vi "process.vi"(8 "error in":errorcluster, 9 "result allocation":T1, 10 "parameters":T1, 11 "module in":refnum<class "alarms module runtime.lvclass">) -> (0 "error out":errorcluster, 1 "results":T1, 2 "parameter allocation":T1, 3 "module out":refnum<class "alarms module runtime.lvclass">)   [LabVIEW 2013, in "alarms module runtime.lvclass"]
doc: "Provides an interface for information processing by a module at runtime. While this interface performs no operations, a child should provide an override which may process data in any manner necessary."
uses:
  alarms module runtime.lvclass
  <vilib>/NI/Tag Bus/table/data table.lvlib
  <vilib>/NI/Tag Bus/table/data polymorphs/read one/read Boolean.vi
  <vilib>/NI/Tag Bus/table/data polymorphs/write one/write Boolean.vi
  <vilib>/NI/Tag Bus/table/data polymorphs/read one/read Single.vi
  <vilib>/NI/Tag Bus/table/data polymorphs/read one/read Double.vi
  <vilib>/NI/Tag Bus/table/data polymorphs/read one/read I64.vi
  <vilib>/NI/Tag Bus/table/data polymorphs/read one/read I32.vi
  <vilib>/NI/Tag Bus/table/data polymorphs/read one/read I16.vi
  <vilib>/NI/Tag Bus/table/data polymorphs/read one/read I8.vi
  <vilib>/NI/Tag Bus/table/data polymorphs/read one/read U64.vi
  <vilib>/NI/Tag Bus/table/data polymorphs/read one/read U32.vi
  <vilib>/NI/Tag Bus/table/data polymorphs/read one/read U16.vi
  <vilib>/NI/Tag Bus/table/data polymorphs/read one/read U8.vi
  <vilib>/NI/Tag Bus/table/data table.ctl
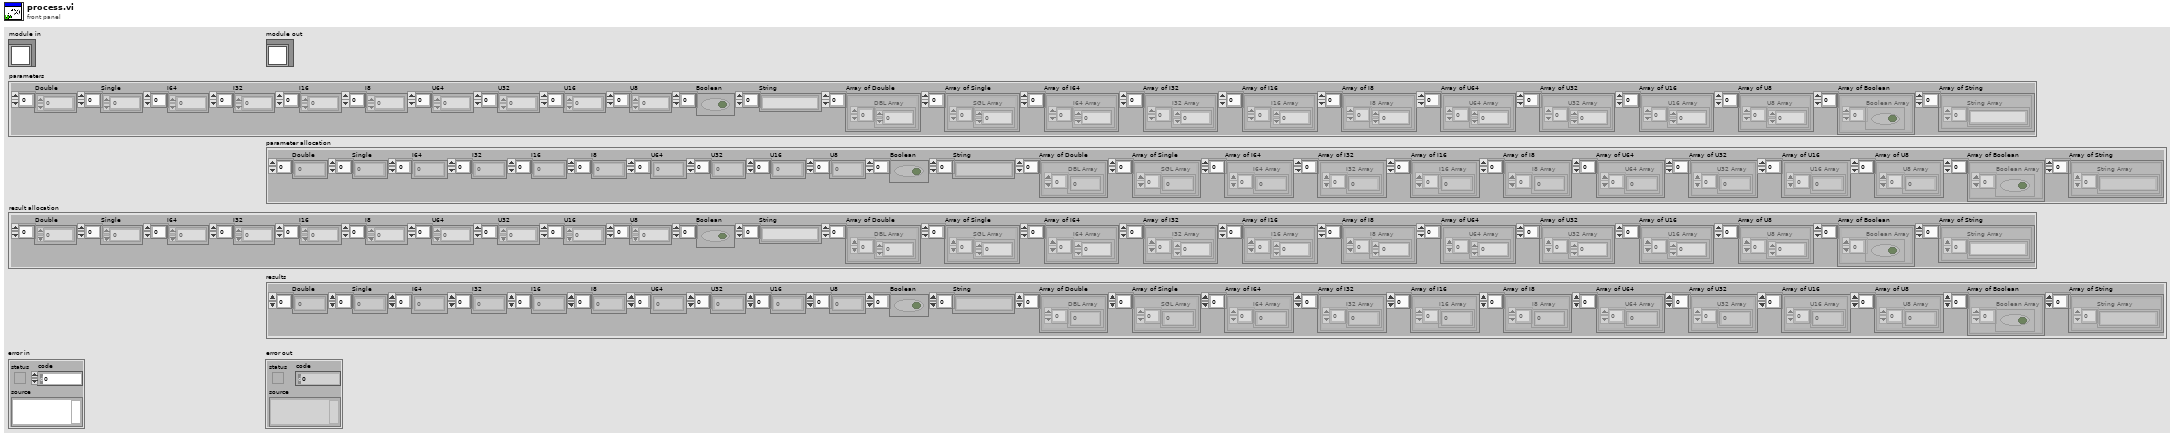
[diagram p1: front panel]
types:
  T1 = typedef "tag bus.lvlib/data table.lvlib/data table.ctl" = cluster{"Double":dbl[], "Single":sgl[], "I64":i64[], "I32":i32[], "I16":i16[], "I8":i8[], "U64":u64[], "U32":u32[], "U16":u16[], "U8":u8[], "Boolean":bool[], "String":string[], "Array of Double":cluster{"DBL Array":dbl[]}[], "Array of Single":cluster{"SGL Array":sgl[]}[], "Array of I64":cluster{"I64 Array":i64[]}[], "Array of I32":cluster{"I32 Array":i32[]}[], "Array of I16":cluster{"I16 Array":i16[]}[], "Array of I8":cluster{"I8 Array":i8[]}[], "Array of U64":cluster{"U64 Array":u64[]}[], "Array of U32":cluster{"U32 Array":u32[]}[], "Array of U16":cluster{"U16 Array":u16[]}[], "Array of U8":cluster{"U8 Array":u8[]}[], "Array of Boolean":cluster{"Boolean Array":bool[]}[], "Array of String":cluster{"String Array":string[]}[]}
  T2 = typedef "alarms module runtime.lvclass/runtime alarm configuration.ctl" = cluster{"comparisons":T3[], "boolean op":T6, "unlatch index (bool)":i32, "output index (bool)":i32, "state":bool}
  T3 = typedef "alarms module runtime.lvclass/runtime alarm comparison.ctl" = cluster{"data type":T4, "index":i32, "limit":dbl, "comparison":T5}
  T4 = typedef "tag bus.lvlib/tag descriptor.lvclass/Data Type.ctl" = enum16{"Double", "Single", "I64", "I32", "I16", "I8", "U64", "U32", "U16", "U8", "Boolean", "String", "Array of Double", "Array of Single", "Array of I64", "Array of I32", "Array of I16", "Array of I8", "Array of U64", "Array of U32", "Array of U16", "Array of U8", "Array of Boolean", "Array of String"}
  T5 = typedef "alarms module configuration.lvclass/compare type.ctl" = enum16{">", "<", ">=", "<=", "="}
  T6 = typedef "alarms module configuration.lvclass/boolean operation.ctl" = enum16{"AND", "OR"}
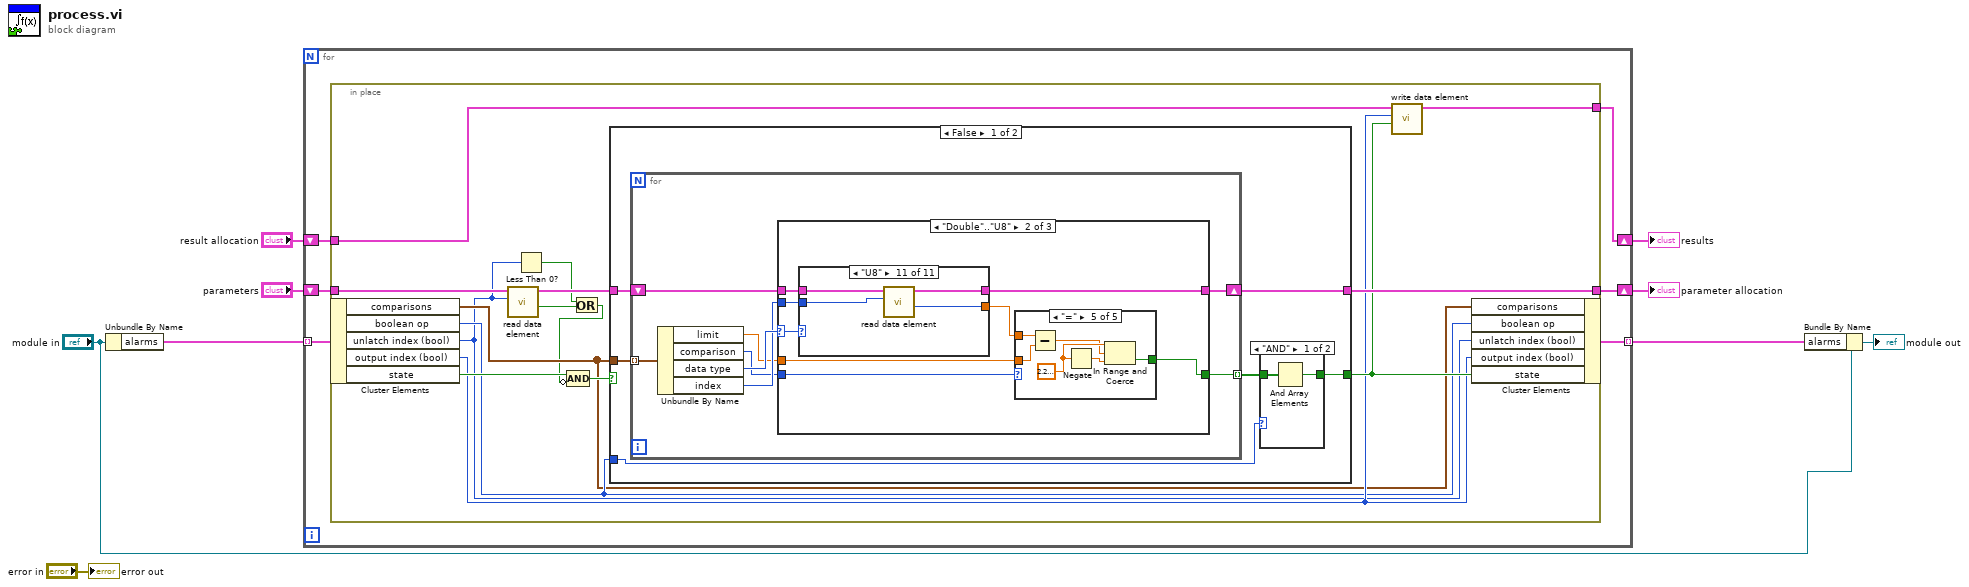
[diagram p0: block diagram]
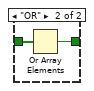
[diagram p2: hidden frame]
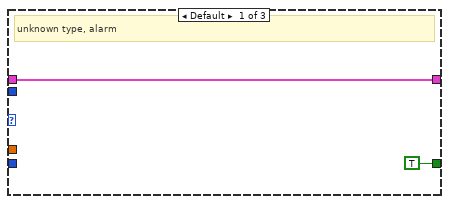
[diagram p3: hidden frame]
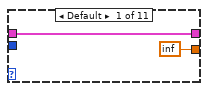
[diagram p4: hidden frame]
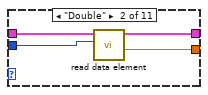
[diagram p5: hidden frame]
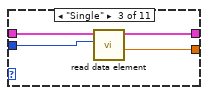
[diagram p6: hidden frame]
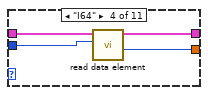
[diagram p7: hidden frame]
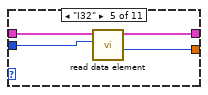
[diagram p8: hidden frame]
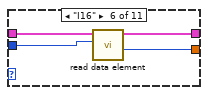
[diagram p9: hidden frame]
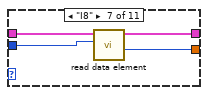
[diagram p10: hidden frame]
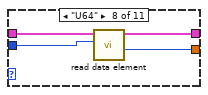
[diagram p11: hidden frame]
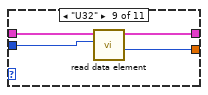
[diagram p12: hidden frame]
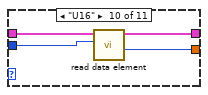
[diagram p13: hidden frame]
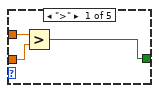
[diagram p14: hidden frame]
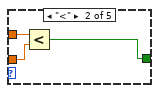
[diagram p15: hidden frame]
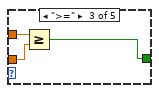
[diagram p16: hidden frame]
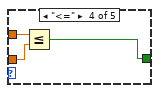
[diagram p17: hidden frame]
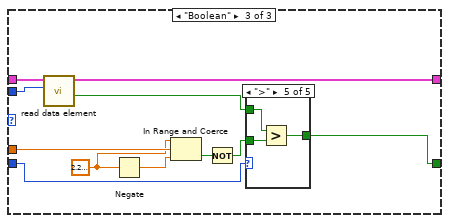
[diagram p18: hidden frame]
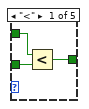
[diagram p19: hidden frame]
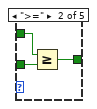
[diagram p20: hidden frame]
diagram:
  n1 = Unbundle By Name("module in") -> ("alarms"=w7:T2[])
  n2 = for {
    tunnel: w7 -> [w15] mode=indexing
    tunnel: [w14] -> w6 mode=indexing
    shift-right: [w12] -> w4
    shift-left: "parameters" -> [w13]
    shift-right: [w10] -> w2
    shift-left: "result allocation" -> [w11]
    n3 = in-place {
      in-place-border: w13 -> [w30]
      in-place-border: [w27] -> w12
      in-place-border: w11 -> [w26]
      in-place-border: [w25] -> w10
      n4 = in-place-cluster #1(w15) -> ("comparisons"=w20:T3[], "boolean op"=w21:T6, "unlatch index (bool)"=w19:i32, "output index (bool)"=w22:i32, "state"=w24:bool)
      n5 = call-poly <vilib>:"read data element.vi"("index"=w19, "data table in"=w30) -> ("value"=w18:bool, "data table out"=w28:T1)  [unwired: 8 in]
      n6 = Less Than 0?(x=w19) -> (x < 0?=w17:bool)
      n7 = Or(x=w17, y=w18) -> (x .or. y?=w16:bool)
      n8 = Compound Arithmetic op=AND(w24, invert w16) -> (w29:bool)
      n9 = case shown="False" w29 {
        selector: w29 -> [_ w145]
        tunnel: w28 -> [w35 w146]
        tunnel: [w34 w146] -> w27
        tunnel: [w32 w145] -> w23
        tunnel: w21 -> [w33 _]
        tunnel: w20 -> [w36 _]
        frame False {
          n10 = for {
            tunnel: w36 -> [w48] mode=indexing
            shift-right: [w45] -> w34
            shift-left: w35 -> [w46]
            tunnel: [w44] -> w31 mode=indexing
            n11 = Unbundle By Name(w48) -> ("limit"=w42:dbl, "comparison"=w41:T5, "data type"=w47:T4, "index"=w43:i32)
            n12 = case shown="\"Double\"..\"U8\"" w47 {
              selector: w47 -> [_ w51 _]
              tunnel: w46 -> [w50 w58 w129]
              tunnel: [w50 w56 w127] -> w45
              tunnel: [TRUE w54 w119] -> w44
              tunnel: w43 -> [_ w57 w128]
              tunnel: w42 -> [_ w52 w126]
              tunnel: w41 -> [_ w55 w122]
              frame Default {
                # "unknown type, alarm"
              }
              frame "Double".."U8" {
                n13 = case shown="\"U64\"" w51 {
                  tunnel: w58 -> [w59 w64 w68 w72 w76 w80 w84 w88 w92 w96 w100]
                  tunnel: w57 -> [_ w63 w67 w71 w75 w79 w83 w87 w91 w95 w99]
                  tunnel: [w59 w62 w66 w70 w74 w78 w82 w86 w90 w94 w98] -> w56
                  tunnel: [inf w61 w65 w69 w73 w77 w81 w85 w89 w93 w97] -> w53
                  frame Default {
                  }
                  frame "Double" {
                    n14 = call-poly <vilib>:"read data element.vi"("index"=w63, "data table in"=w64) -> ("value"=w61:dbl, "data table out"=w62:T1)  [unwired: 8 in]
                  }
                  frame "Single" {
                    n15 = call-poly <vilib>:"read data element.vi"("index"=w67, "data table in"=w68) -> ("value"=w65:sgl, "data table out"=w66:T1)  [unwired: 8 in]
                  }
                  frame "I64" {
                    n16 = call-poly <vilib>:"read data element.vi"("index"=w71, "data table in"=w72) -> ("value"=w69:i64, "data table out"=w70:T1)  [unwired: 8 in]
                  }
                  frame "I32" {
                    n17 = call-poly <vilib>:"read data element.vi"("index"=w75, "data table in"=w76) -> ("value"=w73:i32, "data table out"=w74:T1)  [unwired: 8 in]
                  }
                  frame "I16" {
                    n18 = call-poly <vilib>:"read data element.vi"("index"=w79, "data table in"=w80) -> ("value"=w77:i16, "data table out"=w78:T1)  [unwired: 8 in]
                  }
                  frame "I8" {
                    n19 = call-poly <vilib>:"read data element.vi"("index"=w83, "data table in"=w84) -> ("value"=w81:i8, "data table out"=w82:T1)  [unwired: 8 in]
                  }
                  frame "U64" {
                    n20 = call-poly <vilib>:"read data element.vi"("index"=w87, "data table in"=w88) -> ("value"=w85:u64, "data table out"=w86:T1)  [unwired: 8 in]
                  }
                  frame "U32" {
                    n21 = call-poly <vilib>:"read data element.vi"("index"=w91, "data table in"=w92) -> ("value"=w89:u32, "data table out"=w90:T1)  [unwired: 8 in]
                  }
                  frame "U16" {
                    n22 = call-poly <vilib>:"read data element.vi"("index"=w95, "data table in"=w96) -> ("value"=w93:u16, "data table out"=w94:T1)  [unwired: 8 in]
                  }
                  frame "U8" {
                    n23 = call-poly <vilib>:"read data element.vi"("index"=w99, "data table in"=w100) -> ("value"=w97:u8, "data table out"=w98:T1)  [unwired: 8 in]
                  }
                }
                n24 = case shown="\"<\"" w55 {
                  tunnel: w52 -> [w102 w105 w108 w111 w117]
                  tunnel: w53 -> [w103 w106 w109 w112 w118]
                  tunnel: [w101 w104 w107 w110 w113] -> w54
                  frame ">" {
                    n25 = Greater?(x=w103, y=w102) -> (0:w101:bool)
                  }
                  frame "<" {
                    n26 = Less?(x=w106, y=w105) -> (x < y?=w104:bool)
                  }
                  frame ">=" {
                    n27 = Greater Or Equal?(x=w109, y=w108) -> (x >= y?=w107:bool)
                  }
                  frame "<=" {
                    n28 = Less Or Equal?(x=w112, y=w111) -> (x <= y?=w110:bool)
                  }
                  frame "=" {
                    w115 = 2.220446049250313e-16
                    n29 = Subtract(x=w118, y=w117) -> (x-y=w114:dbl)
                    n30 = Negate(x=w115) -> (-x=w116:dbl)
                    n31 = In Range and Coerce(upper limit=w115, x=w114, lower limit=w116) -> (In Range?=w113:bool)  [unwired: 1 out]
                  }
                }
              }
              frame "Boolean" {
                w124 = 2.220446049250313e-16
                n32 = call-poly <vilib>:"read data element.vi"("index"=w128, "data table in"=w129) -> ("value"=w120:bool, "data table out"=w127:T1)  [unwired: 8 in]
                n33 = Negate(x=w124) -> (-x=w125:dbl)
                n34 = In Range and Coerce(upper limit=w124, x=w126, lower limit=w125) -> (In Range?=w123:bool)  [unwired: 1 out]
                n35 = Not(x=w123) -> (.not. x?=w121:bool)
                n36 = case shown="\">\"" w122 {
                  tunnel: w121 -> [w132 w135 w138 w141 w144]
                  tunnel: w120 -> [w131 w134 w137 w140 w143]
                  tunnel: [w130 w133 w136 w139 w142] -> w119
                  frame "<" {
                    n37 = Less?(x=w131, y=w132) -> (x < y?=w130:bool)
                  }
                  frame ">=" {
                    n38 = Greater Or Equal?(x=w134, y=w135) -> (x >= y?=w133:bool)
                  }
                  frame "<=" {
                    n39 = Less Or Equal?(x=w137, y=w138) -> (x <= y?=w136:bool)
                  }
                  frame "=" {
                    n40 = Equal?(x=w140, y=w141) -> (x = y?=w139:bool)
                  }
                  frame ">" {
                    n41 = Greater?(x=w143, y=w144) -> (0:w142:bool)
                  }
                }
              }
            }
          }
          n42 = case shown="\"AND\"" w33 {
            tunnel: [w38 w40] -> w32
            tunnel: w31 -> [w37 w39]
            frame "AND" {
              n43 = And Array Elements(Boolean array=w37) -> (logical AND=w38:bool)
            }
            frame "OR" {
              n44 = Or Array Elements(Boolean array=w39) -> (logical OR=w40:bool)
            }
          }
        }
        frame True {
          # "already set and NOT unset"
        }
      }
      n45 = call-poly <vilib>:"write data element.vi"("value"=w23, "index"=w22, "data table in"=w26) -> ("data table out"=w25:T1)  [unwired: 8 in]
      n46 = in-place-cluster #1("comparisons"=w20, "boolean op"=w21, "unlatch index (bool)"=w19, "output index (bool)"=w22, "state"=w23) -> (w14:T2)
    }
  }
  "results" <- w2
  "parameter allocation" <- w4
  n47 = Bundle By Name(cluster="module in", "alarms"=w6) -> (→"module out":refnum<class "alarms module runtime.lvclass">)
  "error out" <- "error in"
